vi "Increment.vi"(6 "Labels":map{string, string}(c390), 8 "error in (no error)":errorcluster, 10 "Step":dbl=1.0, 11 "Gauge Ref":refnum<data-value>) -> (0 "error out":errorcluster, 3 "Gauge Ref out":refnum<data-value>)   [LabVIEW 2020, in "Metrics.lvlib" / "Gauge.lvclass"]
doc: "Increments the value of the gauge metric."
uses:
  Gauge.lvclass
  C:/Github-locals/PromVIEW/src/metrics/metric/Metric.lvclass
  <vilib>/Utility/miscctls.llb/LVMapReplaceAction.ctl
  sample/Sample.lvclass/Sample.ctl
  metric/Metric.lvclass/Metric.ctl
  sample/Read Value.vi
  sample/Write Value.vi
  metric/Write Samples 2.vi
  metric/Metric.lvclass
  sample/Sample.lvclass
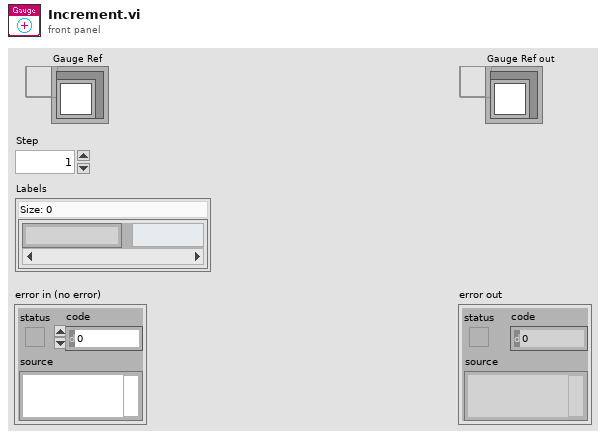
[diagram p1: front panel]
types:
  T1 = typedef "LVMapReplaceAction.ctl" = enum32{"Modify Entry only if found", "Add or Modify Entry", "Delete Entry"}
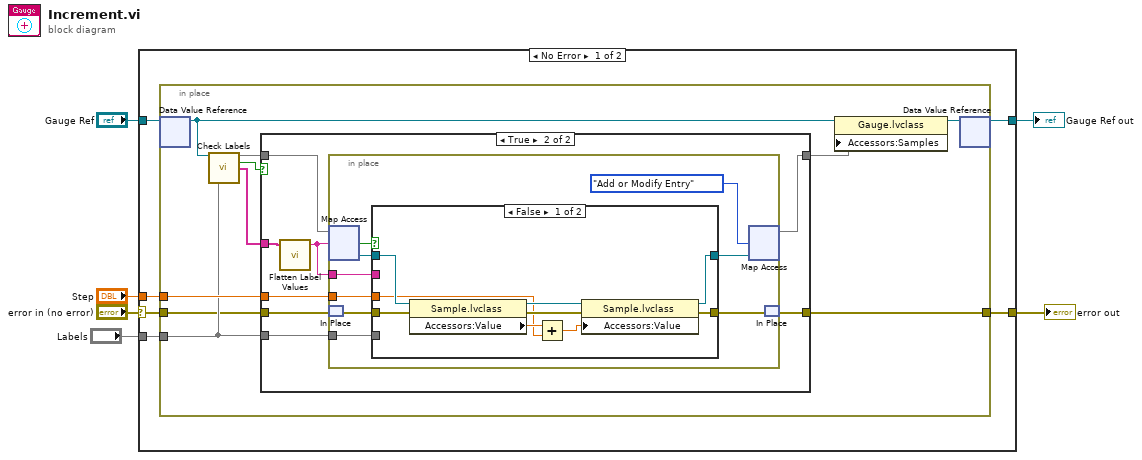
[diagram p0: block diagram]
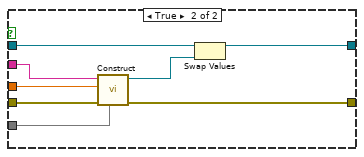
[diagram p3: hidden frame]
diagram:
  n1 = case shown="No Error" "error in (no error)" {
    selector: "error in (no error)" -> [w8 w59]
    tunnel: [w7 w59] -> w5
    tunnel: "Gauge Ref" -> [w12 _]
    tunnel: "Step" -> [w11 _]
    tunnel: "Labels" -> [w10 _]
    tunnel: [w9 _] -> w1
    frame No Error {
      n2 = in-place {
        in-place-border: w11 -> [w19]
        in-place-border: w10 -> [w18]
        in-place-border: w8 -> [w17]
        in-place-border: [w13] -> w7
        n3 = in-place-dvr #1(w12) -> (w16:refnum<class "Gauge.lvclass">)  [unwired: 1 out]
        n4 = call-dynamic "Check Labels.vi"("Metric in"=w16, "Labels"=w18) -> ("Samples"=w22:map{string, refnum<class "Sample.lvclass">}, "Valid Labels"=w21:bool, "Label Values"=w20:string[])  [unwired: 10 in, 1 out]
        n5 = case shown="True" w21 {
          tunnel: w22 -> [w24 w28]
          tunnel: [w24 w31] -> w15
          tunnel: w19 -> [_ w30]
          tunnel: [w23 w29] -> w13
          tunnel: w20 -> [_ w27]
          tunnel: w18 -> [_ w26]
          tunnel: w17 -> [w23 w25]
          frame False {
          }
          frame True {
            n6 = call "Flatten Label Values.vi"("Label Values"=w27) -> ("Flattened labelvalues"=w32:string)  [unwired: 4 in]
            n7 = in-place {
              in-place-border: w32 -> [w39]
              in-place-border: w30 -> [w38]
              in-place-border: w26 -> [w35]
              n8 = in-place-map #2(w28, w32) -> (w37:refnum<class "Sample.lvclass">, w40:bool)  [unwired: 1 in]
              n9 = in-place-match #3(w25) -> (w34:errorcluster)
              n10 = case shown="False" w40 {
                tunnel: [w44 w54] -> w36
                tunnel: w39 -> [_ w58]
                tunnel: w38 -> [w45 w57]
                tunnel: w35 -> [_ w56]
                tunnel: w37 -> [w46 w53]
                tunnel: w34 -> [w43 w52]
                tunnel: [w42 w51] -> w33
                frame False {
                  n11 = property class="Sample.lvclass"(reference=w46, error in=w43) -> (reference out=w50:refnum<class "Sample.lvclass">, error out=w49:errorcluster, "Accessors:Value"=w48:dbl)
                  n12 = Add(x=w48, y=w45) -> (x+y=w47:dbl)
                  n13 = property class="Sample.lvclass"(reference=w50, error in=w49, "Accessors:Value"=w47) -> (reference out=w44:refnum<class "Sample.lvclass">, error out=w42:errorcluster)
                }
                frame True {
                  n14 = call "Construct.vi"("Labels"=w56, "error in (no error)"=w52, "Value"=w57, "Name"=w58) -> ("error out"=w51:errorcluster, "Sample out"=w55:refnum<class "Sample.lvclass">)  [unwired: 6 in]
                  n15 = Swap Values(12:w53, 14:w55) -> (1:w54:refnum<class "Sample.lvclass">)  [unwired: 1 in, 1 out]
                }
              }
              n16 = in-place-map #2(w36, LVMapReplaceAction."Add or Modify Entry" ("action")) -> (w31:map{string, refnum<class "Sample.lvclass">})  [unwired: 2 out]
              n17 = in-place-match #3(w33) -> (w29:errorcluster)
            }
          }
        }
        n18 = property class="Gauge.lvclass"(reference=w16, "Accessors:Samples"=w15) -> (reference out=w14:refnum<class "Gauge.lvclass">)  [unwired: 1 in, 1 out]
        n19 = in-place-dvr #1(w14) -> (w9:refnum<data-value>)  [unwired: 1 out]
      }
    }
    frame Error {
    }
  }
  "error out" <- w5
  "Gauge Ref out" <- w1
